vi "Read Rules.vi"(8 "error in (no error)":errorcluster, 11 "LogFilter In":refnum<class "LogFilter.lvclass">) -> (0 "error out":errorcluster, 2 "Rules":T3={"Global"={"CSM"=[], "LogType"=[], "State"=[], "StateType"=[]}, "CSM"={"LogType"=[], "State"=[], "StateType"=[]}, "PeriodicLog"={"Enable"=FALSE, "Threshold(#/s)"=1.0, "CheckPeriod(s)"=1.0}}, 3 "LogFilter Out":refnum<class "LogFilter.lvclass">)   [LabVIEW 2017, in "Communicable State Machine.lvlib" / "LogFilter.lvclass"]
uses:
  LogFilter.lvclass
  Typedef/_CSM_GlobalLog_MSG_TYPE.ctl
  Typedef/_CSM_GlobalLog_STATE_TYPE.ctl
  LogFilter.lvclass/LogFilter.ctl
  Communicable State Machine.lvlib
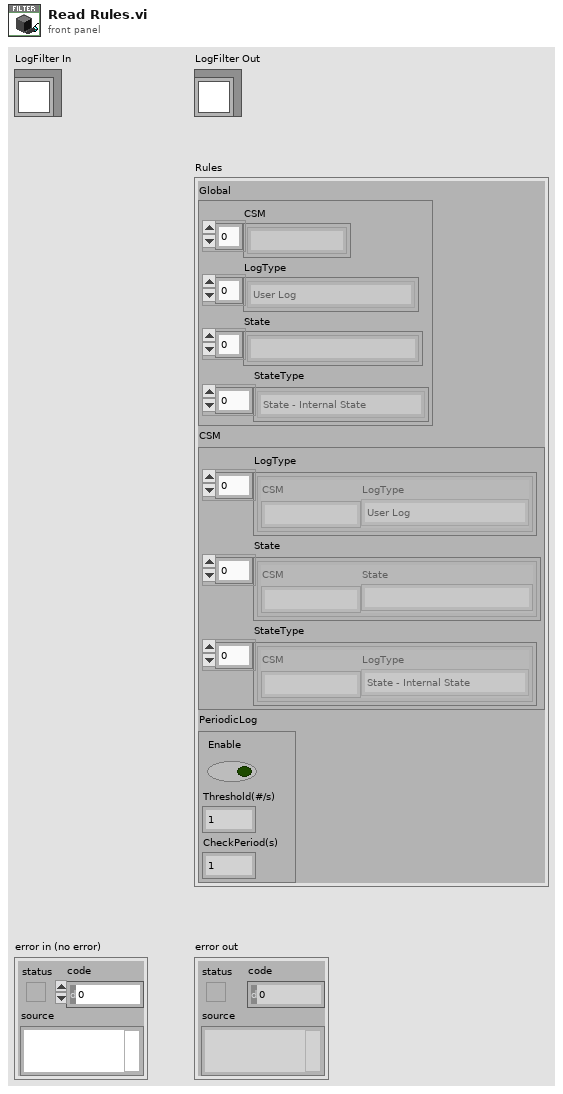
[diagram p1: front panel]
types:
  T1 = typedef "Communicable State Machine.lvlib/_CSM_GlobalLog_MSG_TYPE.ctl" = enum16{"User Log", "State Change", "Status", "Interrupt", "Register", "Unregister", "Error Log", "Module Created", "Module Destroyed"}
  T2 = typedef "Communicable State Machine.lvlib/_CSM_GlobalLog_STATE_TYPE.ctl" = enum16{"State - Internal State", "State - External Message", "State - Response", "State - Complete"}
  T3 = cluster{"Global":cluster{"CSM":string[], "LogType":T1[], "State":string[], "StateType":T2[]}, "CSM":cluster{"LogType":cluster{"CSM":string, "LogType":T1}[], "State":cluster{"CSM":string, "State":string}[], "StateType":cluster{"CSM":string, "LogType":T2}[]}, "PeriodicLog":cluster{"Enable":bool, "Threshold(#/s)":dbl, "CheckPeriod(s)":dbl}}
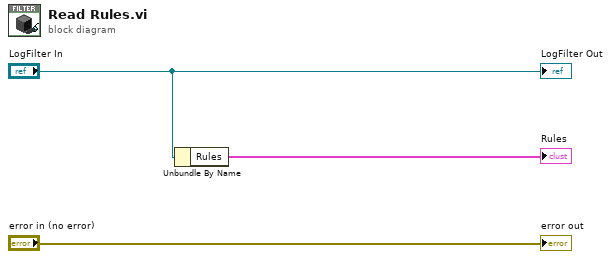
[diagram p0: block diagram]
diagram:
  n1 = Unbundle By Name("LogFilter In") -> ("Rules"=→"Rules":T3)
  "error out" <- "error in (no error)"
  "LogFilter Out" <- "LogFilter In"
